vi "Read All.vi"(6 "Per Read Size":u64=1024 max=30000, 8 "Error In":errorcluster, 10 "Max Read Size":u64=1024, 11 "Channel In":refnum<class "Channel.lvclass">=refnum) -> (0 "Error Out":errorcluster, 1 "Timed Out?":bool, 2 "Data":u8[](array[numeric]), 3 "Channel Out":refnum<class "Channel.lvclass">)   [LabVIEW 2018, in "Toolkit.lvlib" / "Channel.lvclass"]
doc: "Reads binary data from a SSH channel represented by this Channel object in chunks, or blocks, until the total read size is reached. This VI should be used if the <B>Total Read Size</B> is greater than 30KB because of a hard-coded per-read maximum of 30KB set in the libssh2 shared library."
uses:
  Channel.lvclass
  Session/Session.lvclass
  SSH/SSH.lvclass
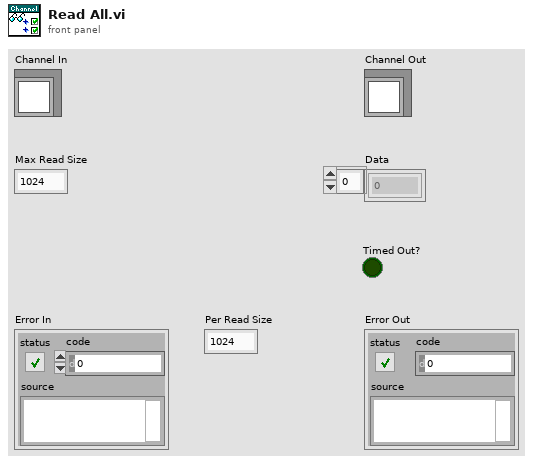
[diagram p1: front panel]
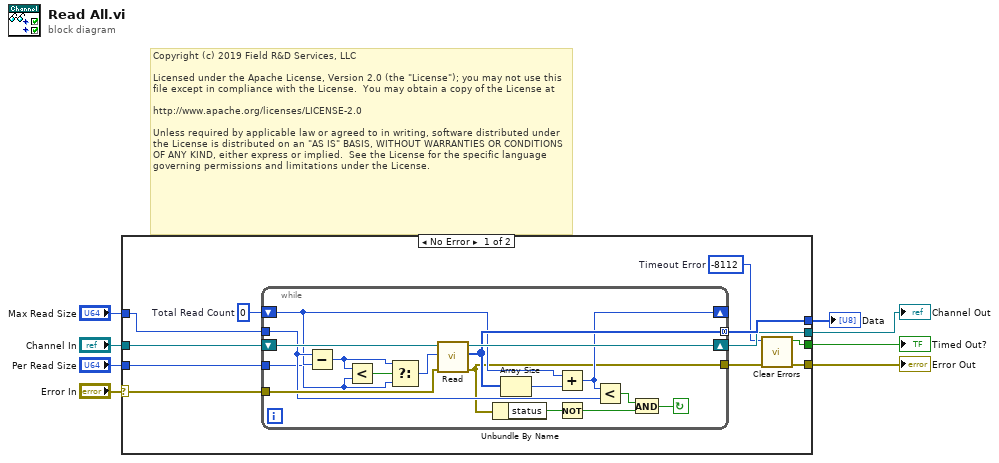
[diagram p0: block diagram]
diagram:
  # "Copyright (c) 2019 Field R&D Services, LLC\n\nLicensed under the Apache License, Version 2.0 (the \"License\"); you may not use this file except in compliance with the License.  You may obtain a copy of the License at\n\nhttp://www.apache.org/licenses/LICENSE-2.0\n\nUnless required by applicable law or agreed to in writing, software distributed under the License is distributed on an \"AS IS\" BASIS, WITHOUT WARRANTIES OR CONDITIONS OF ANY KIND, either express or implied.  See the License for the specific language governing permissions and limitations under the License."
  n1 = case shown="No Error" "Error In" {
    selector: "Error In" -> [w13 w37]
    tunnel: "Max Read Size" -> [w18 _]
    tunnel: "Per Read Size" -> [w17 _]
    tunnel: "Channel In" -> [w16 w38]
    tunnel: [w15 _] -> w5
    tunnel: [w14 w38] -> w4
    tunnel: [w11 w37] -> w3
    tunnel: [w9 _] -> w1
    frame No Error {
      w10 = -8112  # Timeout Error
      w19 = u64 0  # Total Read Count
      n2 = while {
        shift-right: [w34] -> w14
        shift-left: w16 -> [w36]
        tunnel: [w33] -> w15 mode=concatenating
        shift-right: [w31] -> _
        shift-left: w19 -> [w29]
        tunnel: w18 -> [w30]
        tunnel: w17 -> [w25]
        tunnel: w13 -> [w35]
        tunnel: [w24] -> w12
        stop <- w20 continue-if-true
        n3 = Subtract(x=w30, y=w29) -> (x-y=w27:u64)
        n4 = Less?(x=w27, y=w25) -> (x < y?=w28:bool)
        n5 = Select(t=w27, s=w28, f=w25) -> (s? t:f=w26:u64)
        n6 = call "Read.vi"("Error In"=w35, "Max Data Length"=w26, "Channel In"=w36) -> ("Error Out"=w24:errorcluster, "Data"=w33:u8[], "Channel Out"=w34:refnum<class "Channel.lvclass">)  [unwired: 6 in]
        n7 = Unbundle By Name(w24) -> ("status"=w23:bool)
        n8 = Array Size(array=w33) -> (size(s)=w32:i32)
        n9 = Add(x=w29, y=w32) -> (x+y=w31:u64)
        n10 = Not(x=w23) -> (.not. x?=w21:bool)
        n11 = Less?(x=w31, y=w30) -> (x < y?=w22:bool)
        n12 = And(x=w22, y=w21) -> (x .and. y?=w20:bool)
      }
      n13 = call <vilib>:"Clear Errors.vi"("error in (no error)"=w12, "specific error code to clear (0: all)"=w10) -> ("error out"=w11:errorcluster, "specific error cleared?"=w9:bool)  [unwired: 4 in]
    }
    frame Error {
    }
  }
  "Data" <- w5
  "Channel Out" <- w4
  "Error Out" <- w3
  "Timed Out?" <- w1
